vi "GetClassNameW Wrapper Template.vi"(0 "hWnd":u64, 5 "nMaxCount":i32=256, 11 "error in":errorcluster) -> (4 "class name":string, 6 "return value":i32, 15 "error out":errorcluster)   [LabVIEW 2020]
doc: "Returns the class name of the window hWnd through user32.dll GetClassNameW (stdcall, called in any thread), e.g. LVMenuWnd for a LabVIEW ring menu. The buffer is nMaxCount UTF-16 code units of zeros, and the name is cut at its terminating 0 and narrowed code unit by code unit to bytes - exact for ASCII class names, which is what window classes are in practice. return value is the number of characters copied, 0 on failure. When error in carries an error the DLL is not called. Generated by scripts\\Build Win32 Wrappers.vi - do not edit by hand, rebuild it."
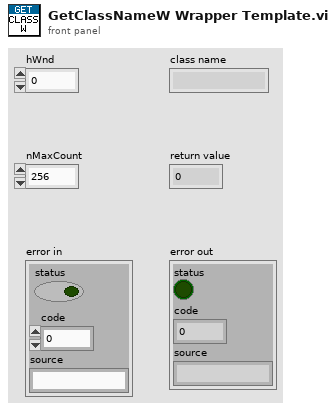
[diagram p1: front panel]
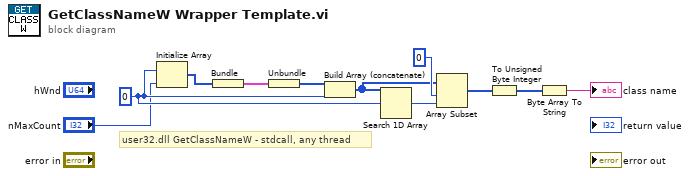
[diagram p0: block diagram]
diagram:
  w3 = u16 0
  # "user32.dll GetClassNameW - stdcall, any thread"
  n1 = Initialize Array(w3, "nMaxCount") -> (w4:u16[])
  n2 = Bundle(w4) -> (w5:cluster{u16[]})  [unwired: 1 in]
  n3 = Unbundle(w5) -> (w6:u16[])
  n4 = Build Array (concatenate)(w6, w3) -> (w7:u16[])
  n5 = Search 1D Array(1D array=w7, element=w3) -> (index of element=w8:i32)  [unwired: 1 in]
  n6 = Array Subset(array=w7, index=0, length=w8) -> (w10:u16[])
  n7 = To Unsigned Byte Integer(number=w10) -> (unsigned 8bit integer=w11:u8[])
  n8 = Byte Array To String(unsigned byte array=w11) -> (string=→"class name":string)
